vi "Explore to Path.vi"(8 "error in (no error)":errorcluster, 10 "Select Directory? (F: Open Directory)":bool, 11 "Path":path) -> (0 "error out":errorcluster)   [LabVIEW 2017, in "csm-ui-support.lvlib"]
uses:
  csm-ui-support.lvlib
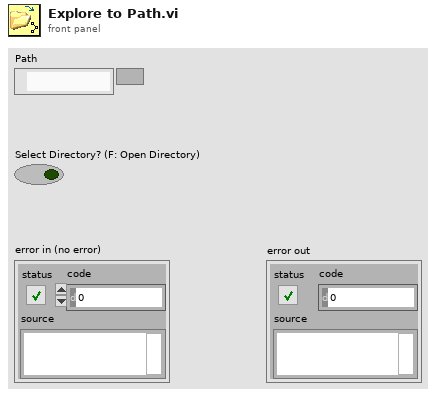
[diagram p1: front panel]
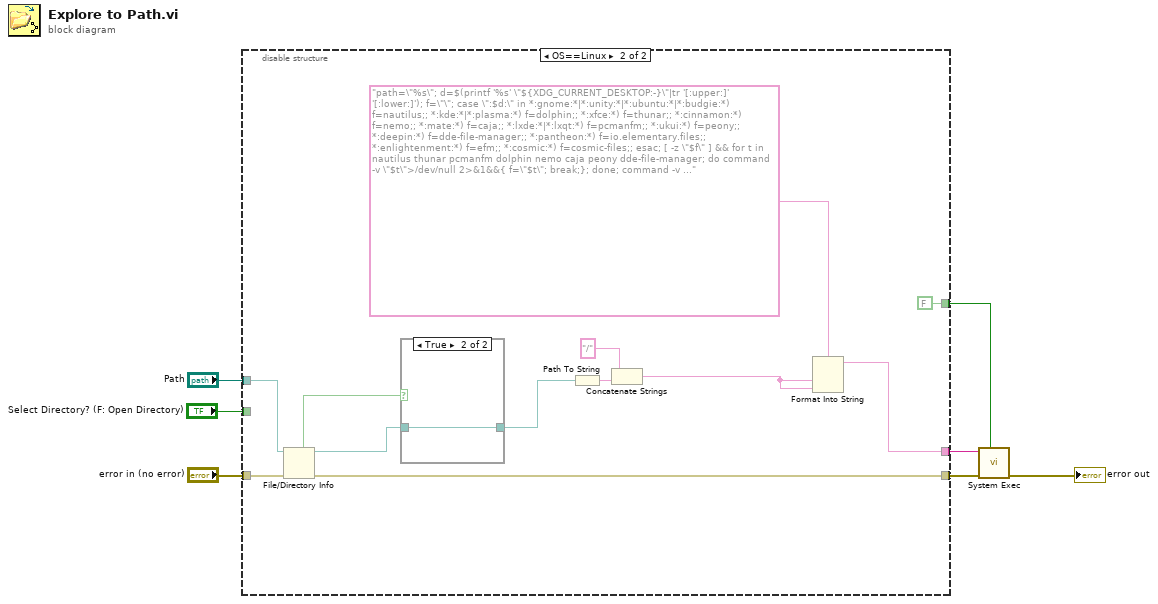
[diagram p0: block diagram]
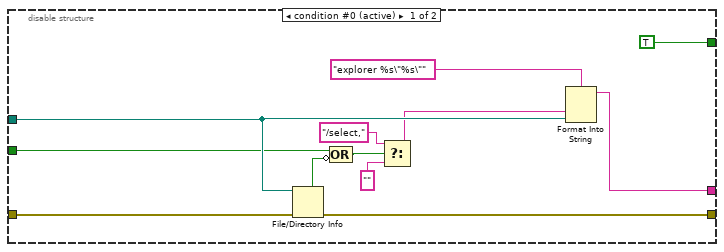
[diagram p2: hidden frame]
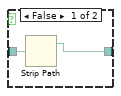
[diagram p3: hidden frame]
diagram:
  n1 = disable-structure shown="OS==Linux" {
    disable-tunnel: "Path" -> [w19 w23]
    disable-tunnel: [w14 w24] -> w5
    disable-tunnel: [w12 w30] -> w4
    disable-tunnel: "error in (no error)" -> [w10 w25]
    disable-tunnel: "Select Directory? (F: Open Directory)" -> [w9 _]
    disable-tunnel: [TRUE ("wait until completion? (T)") FALSE ("wait until completion? (T)")] -> w1
    frame condition #0 (active) {
      n2 = File/Directory Info(path=w19, error in=w10) -> (directory=w13:bool, error out=w14:errorcluster)  [unwired: 5 out]
      n3 = Compound Arithmetic op=OR(w9, invert w13) -> (w15:bool)
      n4 = Select(t="/select," ("format string"), s=w15, f="") -> (s? t:f=w16:string)
      n5 = Format Into String(format string="explorer %s\"%s\"", w16, w19) -> (resulting string=w12:string)  [unwired: 2 in, 1 out]
    }
    frame condition #1 {
      n6 = File/Directory Info(path=w23, error in=w25) -> (path out=w22:path, directory=w21:bool, error out=w24:errorcluster)  [unwired: 4 out]
      n7 = case shown="True" w21 {
        tunnel: w22 -> [w33 w34]
        tunnel: [w32 w34] -> w20
        frame False {
          n8 = Strip Path(path=w33) -> (stripped path=w32:path)  [unwired: 1 out]
        }
        frame True {
        }
      }
      n9 = Path To String(path=w20) -> (string=w27:string)
      n10 = Concatenate Strings("/" ("string"), w27) -> (w26:string)
      n11 = Format Into String(format string="path=\"%s\"; d=$(printf '%s' \"${XDG_CURRENT_DESKTOP:-}\"|tr '[:upper:]' '[:lower:]'); f=\"\"; case \":$d:\" in *:gnome:*|*:unity:*|*:ubuntu:*|*:budgie:*) f=nautilus;; *:kde:*|*:plasma:*) f=dolphin;; *:xfce:*) f=thunar;; *:cinnamon:*) f=nemo;; *:mate:*) f=caja;; *:lxde:*|*:lxqt:*) f=pcmanfm;; *:ukui:*) f=peony;; *:deepin:*) f=dde-file-manager;; *:pantheon:*) f=io.elementary.files;; *:enlightenment:*) f=efm;; *:cosmic:*) f=cosmic-files;; esac; [ -z \"$f\" ] && for t in nautilus thunar pcmanfm dolphin nemo caja peony dde-file-manager; do command -v \"$t\">/dev/null 2>&1&&{ f=\"$t\"; break;}; done; command -v \"$f\">/dev/null 2>&1||f=xdg-open; [ \"$f\" = nautilus ] && nautilus --no-desktop \"$path\" 2>/dev/null||\"$f\" \"$path\"", w26, w26) -> (resulting string=w30:string)  [unwired: 2 in, 1 out]
    }
  }
  n12 = call <vilib>:"System Exec.vi"("wait until completion? (T)"=w1, "error in (no error)"=w5, "command line"=w4) -> ("error out"=→"error out":errorcluster)  [unwired: 5 in, 3 out]
